vi "Open Project Reference.vi"(11 "Test Case In":refnum<class "Runner Unit Test - Add Files to Project.lvclass">) -> (0 "error out":errorcluster, 3 "Test Case Out":refnum<class "Runner Unit Test - Add Files to Project.lvclass">)   [LabVIEW 2026, in "Runner Unit Test - Add Files to Project.lvclass"]
uses:
  Runner Unit Test - Add Files to Project.lvclass
  Runner Unit Test - Add Files to Project.lvclass/Runner Unit Test - Add Files to Project.ctl
  Mocks/Mock IProject Manager/Mock IProject Manager.lvclass
  C:/Program Files/National Instruments/LabVIEW 2026/vi.lib/Astemes/LMock/Mock.lvclass
  C:/Users/juanj/Documents/hasbun_wood_engineering/github/py2vi/labview/Mocks/Mock IProject Manager/Mock IProject Manager.lvclass
  C:/Users/juanj/Documents/hasbun_wood_engineering/github/py2vi/labview/Interfaces/IProject Manager/IProject Manager.lvclass
  Actors/Mock Logger/Mock Logger/Mock Logger.lvclass
  C:/Program Files/National Instruments/LabVIEW 2026/vi.lib/ActorFramework/Actor/Actor.lvclass
  C:/Users/juanj/Documents/hasbun_wood_engineering/github/py2vi/labview/Actors/Mock Logger/Mock Logger/Mock Logger.lvclass
  C:/Users/juanj/Documents/hasbun_wood_engineering/github/py2vi/labview/Interfaces/ILogger/ILogger/ILogger.lvclass
  C:/Program Files/National Instruments/LabVIEW 2026/vi.lib/Astemes/LUnit/Test Case.lvclass
  C:/Program Files/National Instruments/LabVIEW 2026/vi.lib/Astemes/LUnit/LUnit Runnable.lvclass
  C:/Users/juanj/Documents/hasbun_wood_engineering/github/py2vi/labview/Tests/Runner Unit Test - Add Files to Project/Runner Unit Test - Add Files to Project.lvclass
  Actors/Runner/Runner/Runner.lvclass
  Interfaces/IHash Whitelist Handler/IHash Whitelist Handler.lvclass
  Interfaces/ILV File Creator/ILV File Creator.lvclass
  Interfaces/IElement Manager/IElement Manager.lvclass
  Interfaces/IPython Caller/IPython Caller.lvclass
  Interfaces/IFile Manager/IFile Manager.lvclass
  Interfaces/IProject Manager/IProject Manager.lvclass
  Interfaces/IRunner/IRunner/Interfaces--cluster.ctl
  Interfaces/IRunner/IRunner/IRunner.lvclass
  <vilib>/ActorFramework/Actor/Actor.lvclass
  <vilib>/ActorFramework/Stop Msg/Stop Msg.lvclass
  <vilib>/Astemes/LMock/LMock Verifier.lvclass
  <vilib>/Astemes/LMock/LMock.lvlib
  <vilib>/Astemes/LMock/One Identical Inputs.vi
  <vilib>/Astemes/LMock/LMock One.lvlib
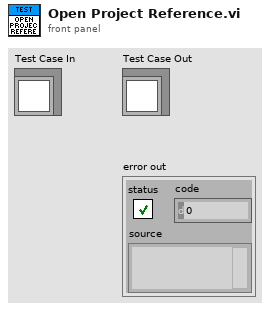
[diagram p1: front panel]
types:
  T1 = typedef "IRunner.lvlib/IRunner.lvclass/Interfaces--cluster.ctl" = cluster{"IProject Manager":refnum<class "IProject Manager.lvclass">, "IFile Manager":refnum<class "IFile Manager.lvclass">, "IPython Caller":refnum<class "IPython Caller.lvclass">, "IElement Manager":refnum<class "IElement Manager.lvclass">, "ILV File Creator":refnum<class "ILV File Creator.lvclass">, "IHash Whitelist Handler":refnum<class "IHash Whitelist Handler.lvclass">}
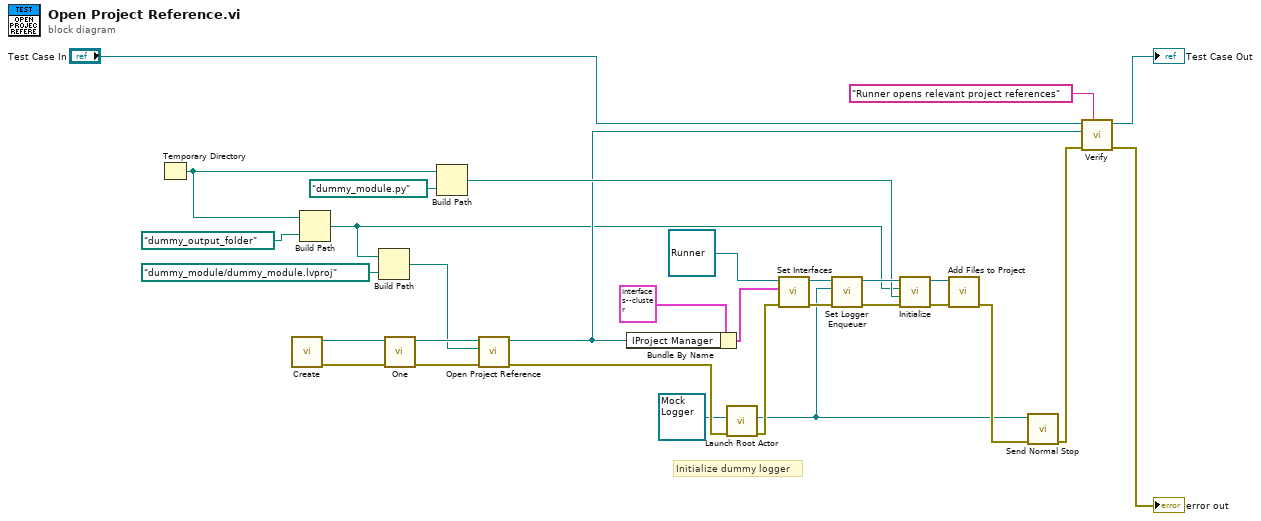
[diagram p0: block diagram]
diagram:
  # "Initialize dummy logger"
  n1 = Temporary Directory() -> (w10:path)
  n2 = call "Create.vi"() -> ("error out"=w24:errorcluster, "Mock Class Generator out"=w6:refnum<class "Mock IProject Manager.lvclass">)  [unwired: 10 in]
  n3 = Build Path(base path=w10, name or relative path=path "dummy_output_folder") -> (appended path=w3:path)
  n4 = Build Path(base path=w3, name or relative path=path "dummy_module/dummy_module.lvproj") -> (appended path=w1:path)
  n5 = call-poly <vilib>:"One.vi"("error in (no error)"=w24, "Mock in"=w6) -> ("error out"=w23:errorcluster, "Mock out"=w5:refnum<class "Mock IProject Manager.lvclass">)  [unwired: 8 in]
  n6 = Build Path(base path=w10, name or relative path=path "dummy_module.py") -> (appended path=w11:path)
  n7 = call-dynamic "Open Project Reference.vi"("error in"=w23, "Path"=w1, "IProject Manager in"=w5) -> ("error out"=w22:errorcluster, "IProject Manager out"=w4:refnum<class "Mock IProject Manager.lvclass">)  [unwired: 7 in]
  n8 = Bundle By Name(cluster=T1 {"IProject Manager"=refnum, "IFile Manager"=refnum, "IPython Caller"=refnum, "IElement Manager"=refnum, "ILV File Creator"=refnum, "IHash Whitelist Handler"=refnum} ("Interfaces"), "IProject Manager"=w4) -> (w18:T1)
  n9 = call <vilib>:"Launch Root Actor.vi"("error in (no error)"=w22, "Actor"=refnum<class "Mock Logger.lvclass"> refnum ("Mock Logger.lvlib:Mock Logger.lvclass")) -> ("error out"=w30:errorcluster, "Actor's Enqueuer"=w16:refnum<class "Message Enqueuer.lvclass">)  [unwired: 8 in]
  n10 = call-dynamic "Set Interfaces.vi"("error in"=w30, "Interfaces"=w18, "Runner in"=refnum<class "Runner.lvclass"> refnum ("Runner.lvlib:Runner.lvclass")) -> ("error out"=w31:errorcluster, "Runner out"=w20:refnum<class "Runner.lvclass">)  [unwired: 7 in]
  n11 = call-dynamic "Set Logger Enqueuer.vi"("error in"=w31, "Logger"=w16, "Runner in"=w20) -> ("error out"=w28:errorcluster, "Runner out"=w13:refnum<class "Runner.lvclass">)  [unwired: 7 in]
  n12 = call-dynamic "Initialize.vi"("error in"=w28, "Python Module"=w11, "Output Folder"=w3, "G-CLI Runner in"=w13) -> ("error out"=w26:errorcluster, "G-CLI Runner out"=w7:refnum<class "Runner.lvclass">)  [unwired: 6 in]
  n13 = call-dynamic "Add Files to Project.vi"("error in"=w26, "Runner in"=w7) -> ("error out"=w25:errorcluster)  [unwired: 8 in, 1 out]
  n14 = call <vilib>:"Send Normal Stop.vi"("error in (no error)"=w25, "Message Enqueuer"=w16) -> ("error out"=w29:errorcluster)  [unwired: 9 in]
  n15 = call <vilib>:"Verify.vi"("Description"="Runner opens relevant project references", "error in (no error)"=w29, "Mock"=w4, "LUnit Test Case In"="Test Case In") -> ("error out"=→"error out":errorcluster, "LUnit Test Case Out"=→"Test Case Out":refnum<class "Runner Unit Test - Add Files to Project.lvclass">)  [unwired: 6 in]
